vi "Update_UI_Test_Sequence.vi"(0 "queue out 2":refnum<queue>, 1 "result":string="Pass", 2 "input cluster":T2={"User name"="", "user account"="", "UI"=[], "DI"=[], "Barcode"="", "MCListbox Ref_in"=refnum, "sequence step #"=0, "Result?"=FALSE, "Report Path"=path "", "Test Sequence"=enum."Ensure all the connections are OK", "skip Test  "=[FALSE, FALSE, FALSE, FALSE, FALSE, FALSE, FALSE, FALSE, FALSE, FALSE, FALSE, FALSE, FALSE, FALSE, FALSE, FALSE, FALSE, FALSE, FALSE, FALSE, FALSE, FALSE, FALSE, FALSE, FALSE, FALSE, FALSE, FALSE, FALSE, FALSE, FALSE, FALSE]} {"DI"."Upper limit" format="%#_7f"; "DI"."Lower limit" format="%#_7f"}, 3 "Result":bool=TRUE, 4 "measured value":string="Started", 5 "error in":errorcluster, 8 "Main Test Status":refnum<vi>) -> (14 "queue out":refnum<queue>, 15 "Main test sequence":T1, 16 "output cluster":T2={"User name"="", "user account"="", "UI"=[], "DI"=[], "Barcode"="", "MCListbox Ref_in"=refnum, "sequence step #"=0, "Result?"=FALSE, "Report Path"=path "", "Test Sequence"=enum."Ensure all the connections are OK", "skip Test  "=[FALSE, FALSE, FALSE, FALSE, FALSE, FALSE, FALSE, FALSE, FALSE, FALSE, FALSE, FALSE, FALSE, FALSE, FALSE, FALSE, FALSE, FALSE, FALSE, FALSE, FALSE, FALSE, FALSE, FALSE, FALSE, FALSE, FALSE, FALSE, FALSE, FALSE, FALSE, FALSE]} {"DI"."Upper limit" format="%#_7f"; "DI"."Lower limit" format="%#_7f"}, 19 "error out":errorcluster)   [LabVIEW 2021]
uses:
  5.ACTIVITIES/1.LabVIEW_State_Machine_Template/LabVIEW_State_Machine_Template/LabVIEW_State_Machine_Template/Project_Template/Queue Test updator/Controls/initialise cluster.ctl
  5.ACTIVITIES/1.LabVIEW_State_Machine_Template/LabVIEW_State_Machine_Template/LabVIEW_State_Machine_Template/Project_Template/Queue Test updator/Controls/test step description.ctl
  5.ACTIVITIES/1.LabVIEW_State_Machine_Template/LabVIEW_State_Machine_Template/LabVIEW_State_Machine_Template/Project_Template/Queue Test updator/Controls/comparison selection.ctl
  controls/Main test sequence.ctl
panel:
  out "UI":string[][](array[string])
  out "Test status item names":string[][](array[string])
  in  "Disable prompt":bool
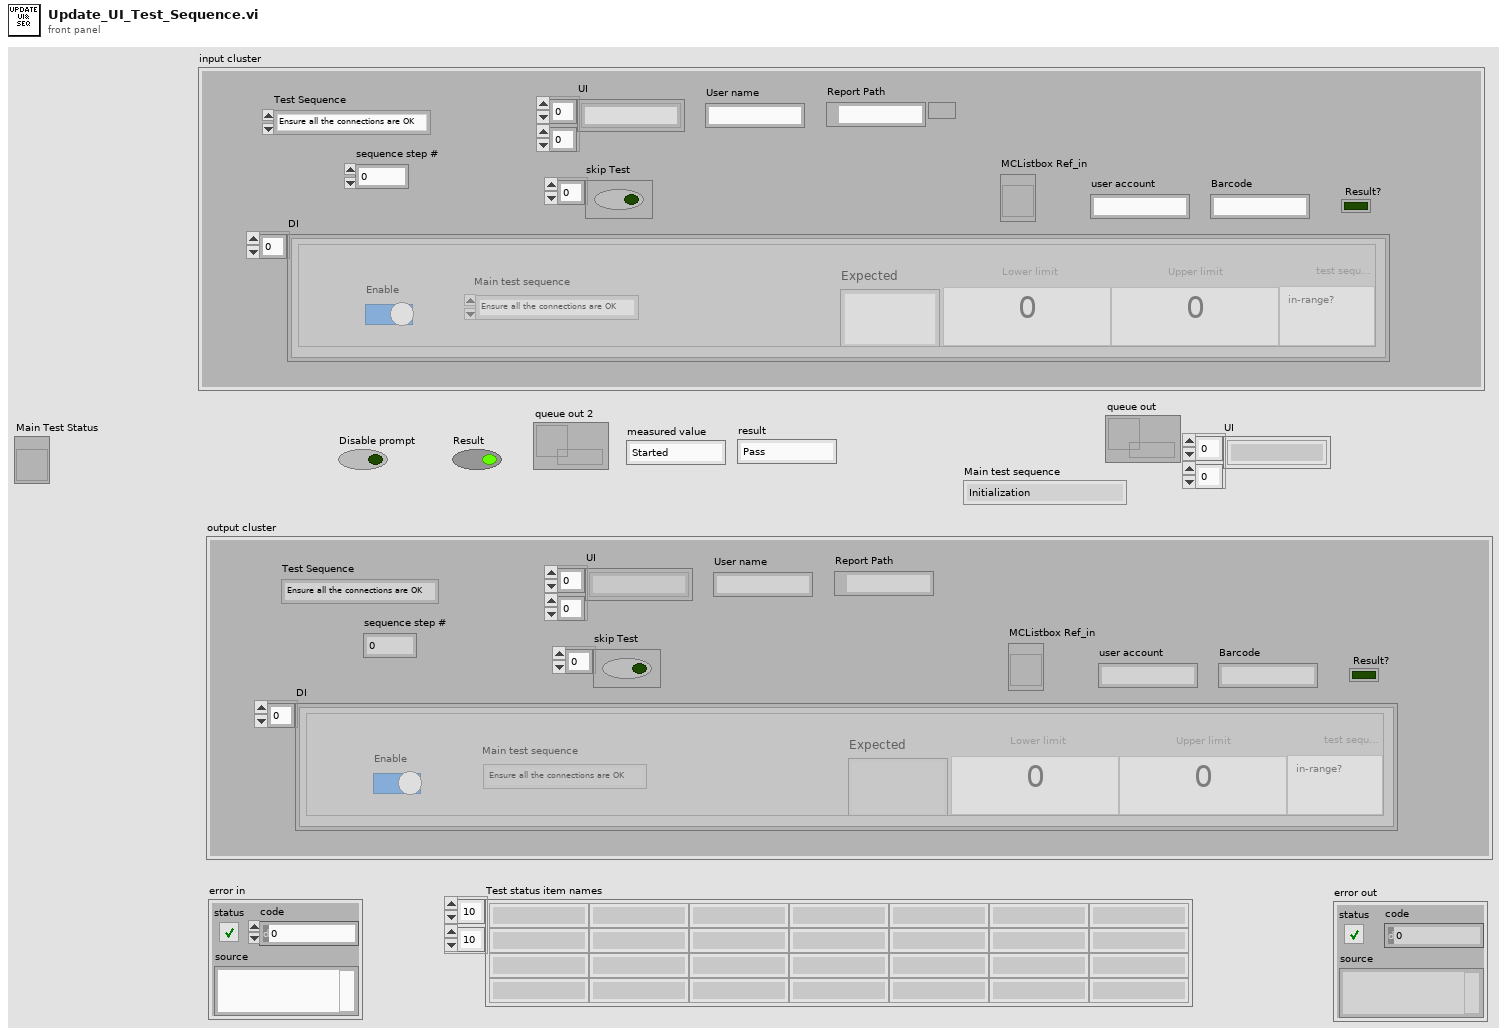
[diagram p1: front panel]
types:
  T1 = typedef "Main test sequence.ctl" = enum16{"Initialization", "Ensure all the connections are OK", "Turn ON 230V AC Input", "Load the Firmware", "Unlock_Opensesame & Stop console Logs", "Earth Detection", "Read Firmware", "Read & Write PCB Serial No", "Emergancy Switch Check", "Update WIFI credentials ", "Reboot", "Unlock Opensesame & Stop_console Logs", "WIFI State", "WIFI SSID", "Board revision", "ADC NTC Temp", "ADC_TYPE2_RCD_CURRENT", "5V Output Voltage", "3.3V Output Voltage", "D+M Sense", "Output Weld Sense", "FW Power Reset", "Unlock Opensesame & Stop console_Logs", "Reset switch Check", "Exit"}
  T2 = typedef "initialise cluster.ctl" = cluster{"User name":string, "user account":string, "UI":string[][], "DI":T3[], "Barcode":string, "MCListbox Ref_in":refnum<vi>, "sequence step #":u32, "Result?":bool, "Report Path":path, "Test Sequence":T1, "skip Test  ":bool[]}
  T3 = typedef "test step description.ctl" = cluster{"Lower limit":dbl, "Upper limit":dbl, "Comparison":T4, "Expected":string, "Enable":bool, "Main test sequence":T1}
  T4 = typedef "comparison selection.ctl" = enum16{"None", "in-range?", "less than?", "greater than?", "equal to?", "not equal to?", "less or equal to?", "greater or equal to?"}
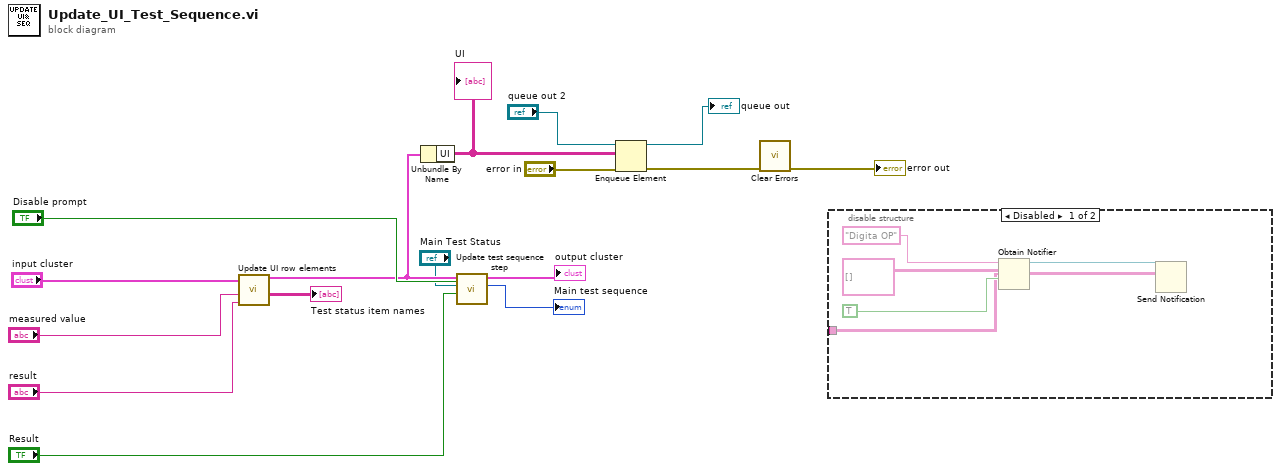
[diagram p0: block diagram]
diagram:
  n1 = call "Update UI row elements.vi"("result"="result", "measured value"="measured value", "input cluster"="input cluster") -> ("Test status item names"=→"Test status item names":string[][], "output cluster"=w5:T2)  [unwired: 7 in]
  n2 = Unbundle By Name(w5) -> ("UI"=w8:string[][])
  "UI" <- w8
  n3 = call "Update test sequence step.vi"("Disable \nprompt"="Disable prompt", "Result"="Result", "Main Test Status"="Main Test Status", "input cluster"=w5) -> ("Main test sequence"=→"Main test sequence":T1, "output cluster"=→"output cluster":T2)  [unwired: 6 in]
  n4 = Enqueue Element(queue="queue out 2", element=w8, error in (no error)="error in") -> (queue out=→"queue out":refnum<queue>, error out=w2:errorcluster)  [unwired: 1 in, 1 out]
  n5 = call <vilib>:"Clear Errors.vi"("error in (no error)"=w2) -> ("error out"=→"error out":errorcluster)  [unwired: 5 in, 1 out]
  n6 = disable-structure shown="Disabled" {
    disable-tunnel: _ -> [w17 _]
    frame Disabled {
      n7 = Obtain Notifier(name (unnamed)="Digita OP", notification data type=string[][] [] ("Test status item names"), create if not found? (T)=TRUE) -> (notifier out=w21:refnum<notifier>)  [unwired: 1 in, 2 out]
      n8 = Send Notification(notification=w17, notifier=w21) -> ()  [unwired: 1 in, 2 out]
    }
    frame Enabled {
    }
  }
